vi "Test Function Generator API.vi"() -> ()   [LabVIEW 2026]
doc: "Function Generator API Tester."
uses:
  <vilib>/Utility/error.llb/DialogType.ctl
  <vilib>/Utility/error.llb/Search and Replace Pattern (string).vi
  Function Generator.lvlib
panel:
  out "Map":map{i32, dbl[]}(c390)
  in  "Stop FGEN":bool
  in  "Start":bool
  in  "amplitude":dbl=1.0 format="%0.2p"
  in  "phase":dbl format="%.2p"
  in  "frequency":dbl=10.0 format="%0.2p"
  in  "offset":dbl format="%0.2p"
  in  "Set Signal Parameters":bool
  in  "signal type":T1(ring)
  in  "Set Signal Type":bool
  out "last error":errorcluster
  in  "Show Diagram on Init":bool
  in  "Run as Singleton?":bool
  in  "Show Block Diagram":bool
  in  "Refresh Modules":bool
  out "Active Modules":string[](array[string])
  in  "Stop Module":bool
  in  "Select Module":i32(ring)=-1 caption="Select Module\nTo send Request to" items=["All"=-1]
  in  "Run New Module":bool
  in  "Hide Module Panel":bool
  in  "Show Module Panel":bool
  out "Status":string
  # "This VI tests the API for the Module."
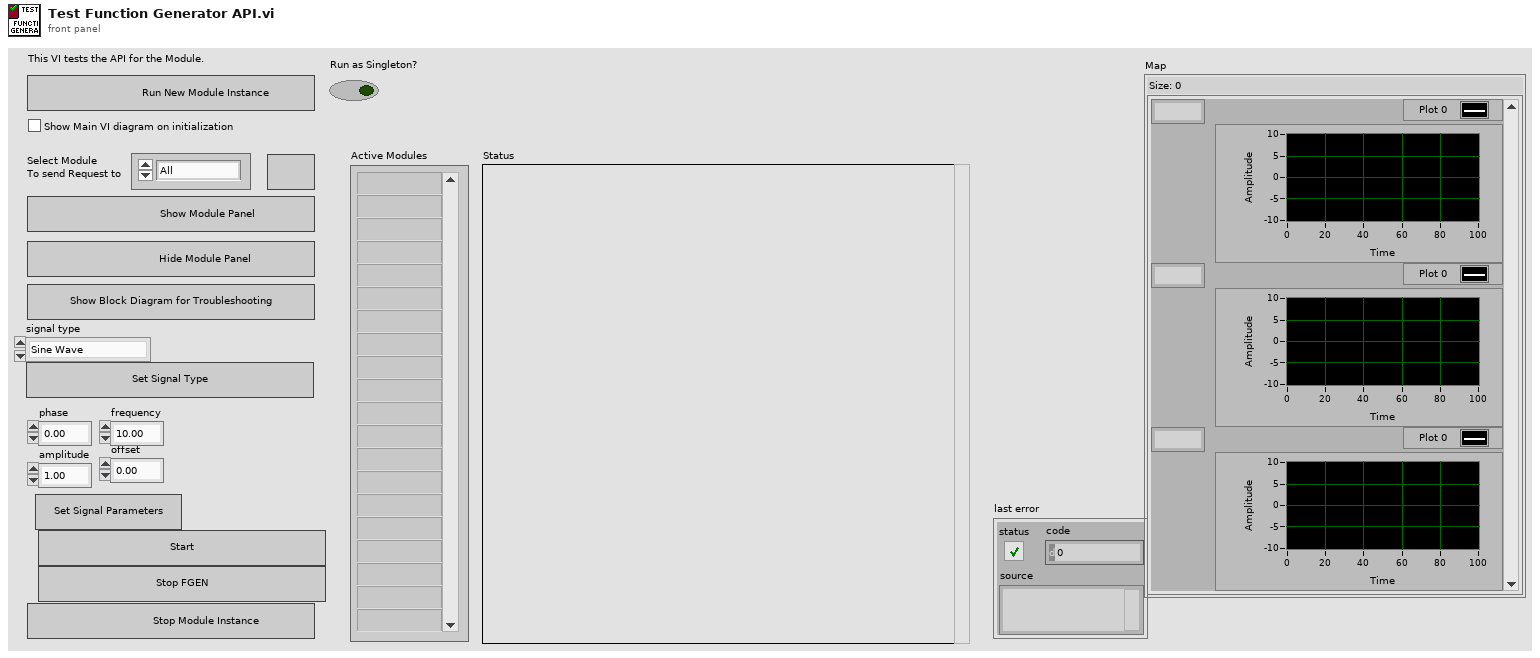
[diagram p1: front panel]
types:
  T1 = enum16{"Sine Wave", "Triangle Wave", "Square Wave", "Sawtooth Wave"}
  T2 = typedef "Function Generator.lvlib/Broadcast Events--cluster.ctl" = cluster{"Module Did Init":refnum<user-event>, "Status Updated":refnum<user-event>, "Error Reported":refnum<user-event>, "Module Did Stop":refnum<user-event>, "Update Module Execution Status":refnum<user-event>, "Waveform Updated":refnum<user-event>}
  T3 = typedef "DialogType.ctl" = u16
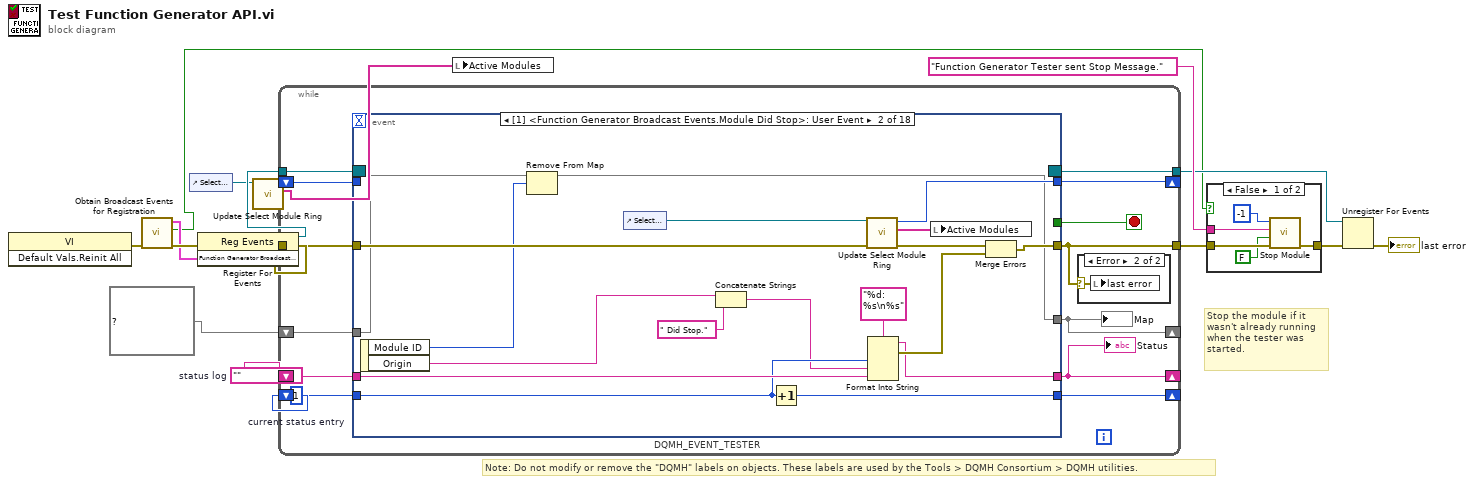
[diagram p0: block diagram]
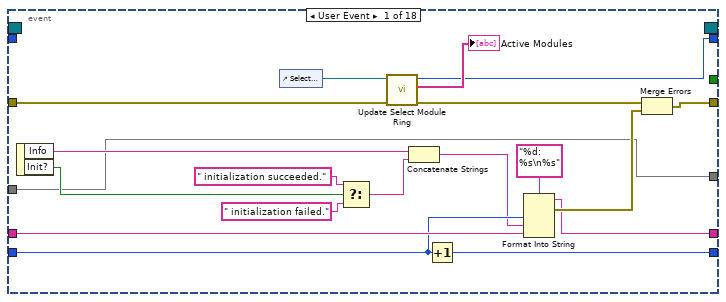
[diagram p4: hidden frame]
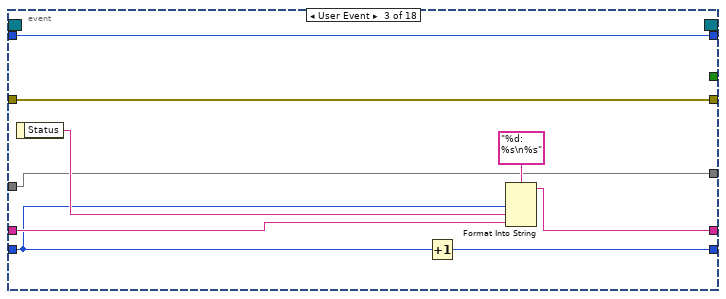
[diagram p5: hidden frame]
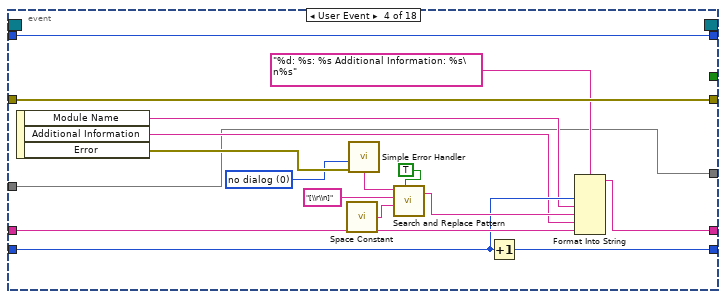
[diagram p6: hidden frame]
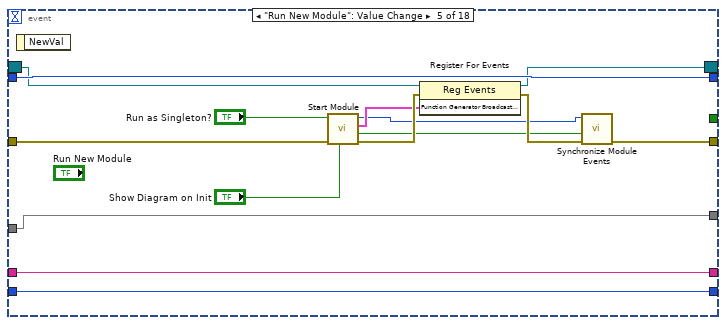
[diagram p7: hidden frame]
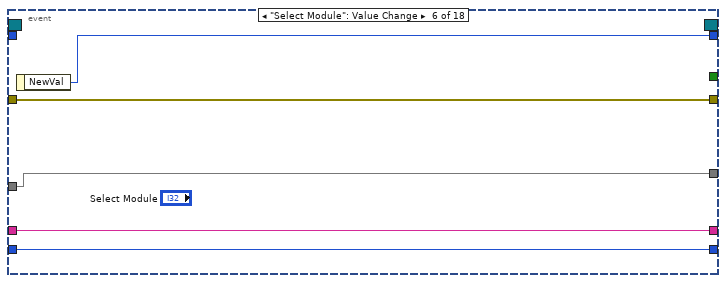
[diagram p8: hidden frame]
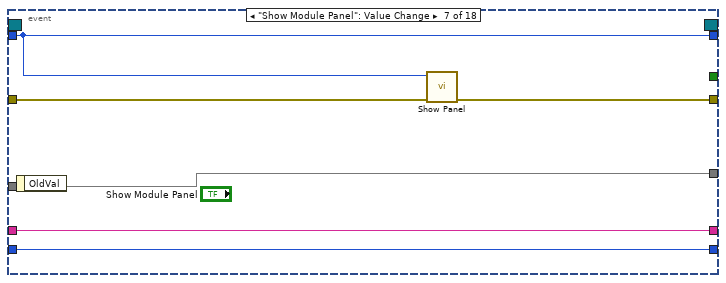
[diagram p9: hidden frame]
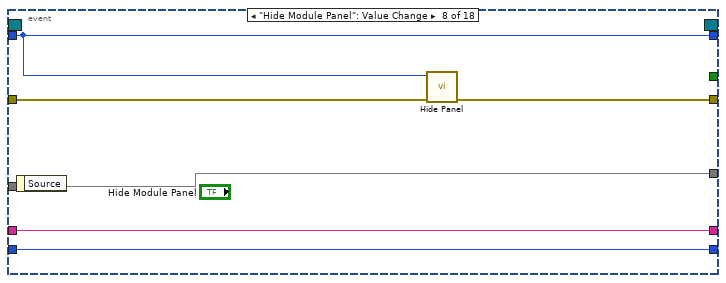
[diagram p10: hidden frame]
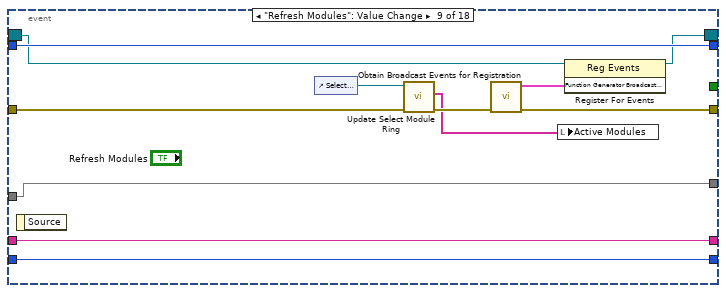
[diagram p11: hidden frame]
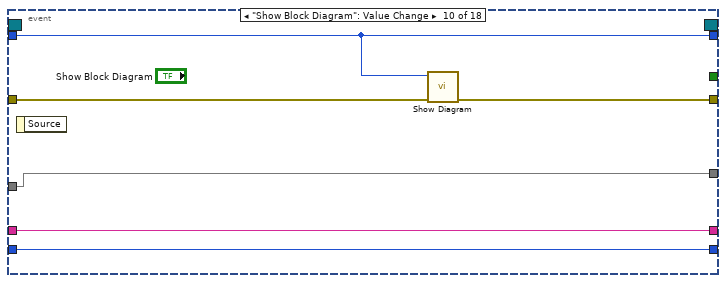
[diagram p12: hidden frame]
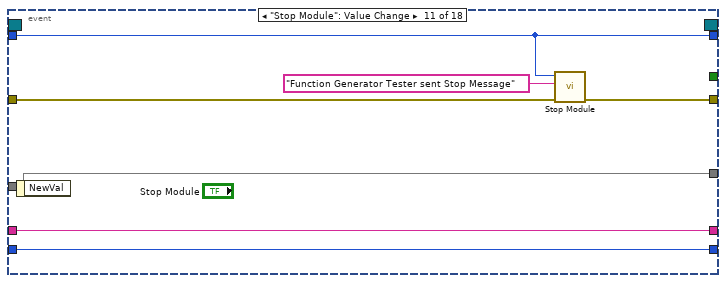
[diagram p13: hidden frame]
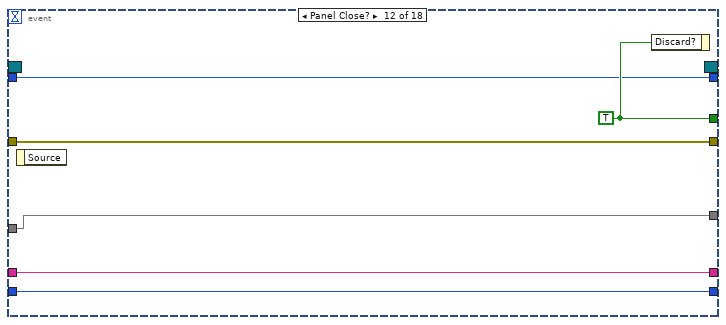
[diagram p14: hidden frame]
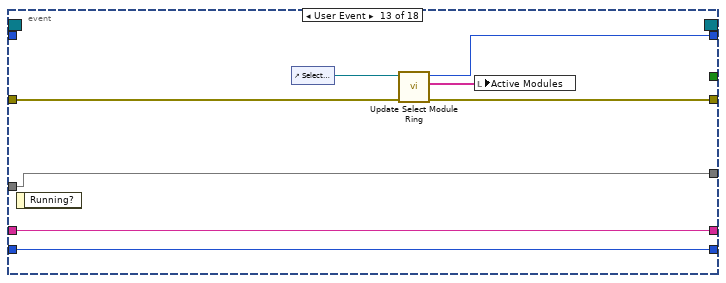
[diagram p15: hidden frame]
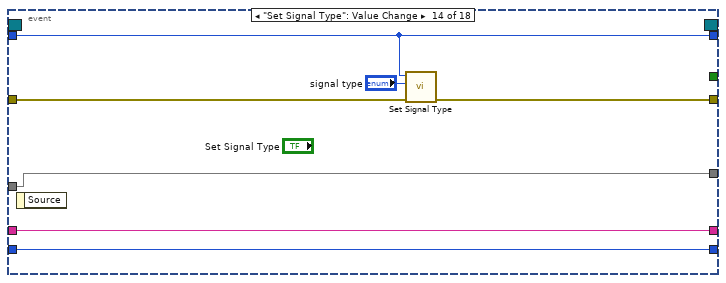
[diagram p16: hidden frame]
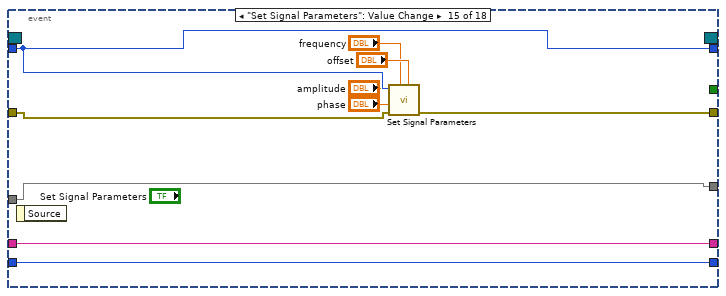
[diagram p17: hidden frame]
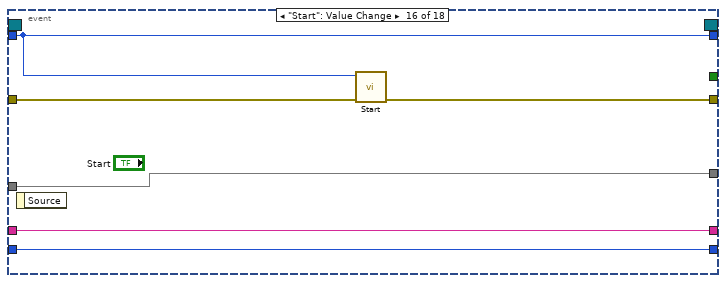
[diagram p18: hidden frame]
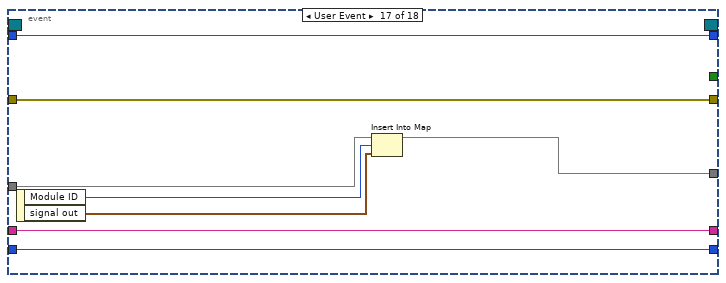
[diagram p19: hidden frame]
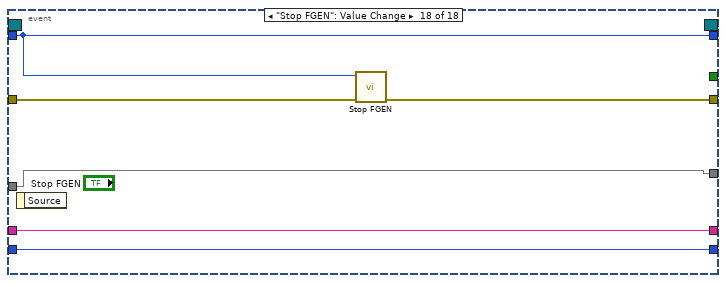
[diagram p20: hidden frame]
diagram:
  w9 = 1  # current status entry
  w10 = ""  # status log
  # "Stop the module if it wasn't already running when the tester was started."
  # "Note: Do not modify or remove the \"DQMH\" labels on objects. These labels are used by the Tools > DQMH Consortium > DQMH utilities."
  n1 = invoke on="Invoke Node" class="VI" method="Default Vals.Reinit All"() -> (error out=w15:errorcluster)  [unwired: 3 in, 2 out]
  n2 = call "Obtain Broadcast Events for Registration.vi"("error in"=w15) -> ("error out"=w14:errorcluster, "Already running?"=w5:bool, "Function Generator Broadcast Events"=w8:T2)  [unwired: 8 in]
  n3 = control-ref of="Select Module"() -> (w4:refnum<vi>)
  n4 = register-events(error in=w14, w8) -> (reference out=w11:refnum<event-registration>, error out=w16:errorcluster)  [unwired: 1 in]
  n5 = call "Update Select Module Ring.vi"("Select Module Ring Ref"=w4) -> ("Active Modules (Array)"=w2:string[], "New Module Ring Value"=w3:i32)  [unwired: 8 in, 1 out]
  n6 = while {
    tunnel: w11 -> [w28]
    tunnel: [w29] -> w13
    tunnel: w16 -> [w30]
    shift-right: [w24] -> _
    shift-left: w10 -> [w26]
    shift-right: [w25] -> _
    shift-left: w9 -> [w27]
    shift-right: [w22] -> _
    shift-left: w3 -> [w23]
    tunnel: [w21] -> w6
    shift-right: [w18] -> _
    shift-left: map{i32, dbl[]} {} ("Map") -> [w19]
    stop <- w20 stop-if-true
    n7 = event "DQMH_EVENT_TESTER" shown="[1] <Function Generator Broadcast Events.Module Did Stop>: User Event" {
      selector: w28 -> [_ _ _ _ w102 _ _ _ w131 _ _ _ _ _ _ _ _ _]
      dyn-events: [_ _ _ _ w101 _ _ _ w130 _ _ _ _ _ _ _ _ _] -> w21
      timeout: _ -> [_ _ _ _ _ _ _ _ _ _ _ _ _ _ _ _ _ _]
      tunnel: [_ _ _ _ _ _ _ _ _ _ _ w156 _ _ _ _ _ _] -> w20
      tunnel: [w47 w65 w77 w94 w106 w114 w119 w125 w136 w143 w150 w157 w164 w171 w181 w187 w196 w201] -> w29
      tunnel: w30 -> [w49 w67 w77 w94 w107 w114 w120 w126 w138 w144 w151 w157 w165 w172 w182 w188 w196 w202]
      tunnel: w27 -> [w44 w62 w70 w83 w104 w112 w117 w123 w134 w141 w148 w154 w162 w169 w179 w185 w193 w199]
      tunnel: w26 -> [w45 w63 w73 w84 w105 w113 w118 w124 w135 w142 w149 w155 w163 w170 w180 w186 w194 w200]
      tunnel: [w42 w60 w74 w82 w105 w113 w118 w124 w135 w142 w149 w155 w163 w170 w180 w186 w194 w200] -> w24
      tunnel: [w43 w61 w76 w81 w104 w112 w117 w123 w134 w141 w148 w154 w162 w169 w179 w185 w193 w199] -> w25
      tunnel: w23 -> [_ _ w71 w92 w103 _ w116 w122 w133 w140 w147 w153 _ w168 w178 w184 w195 w198]
      tunnel: [w37 w57 w71 w92 w103 w111 w116 w122 w133 w140 w147 w153 w160 w168 w178 w184 w195 w198] -> w22
      tunnel: w19 -> [w32 w53 w69 w78 w95 w110 w115 w121 w127 w139 w145 w152 w158 w166 w173 w183 w192 w197]
      tunnel: [w32 w52 w69 w78 w95 w110 w115 w121 w127 w139 w145 w152 w158 w166 w173 w183 w189 w197] -> w18
      event User Event {
        n8 = event-data() -> ("Info"=w41:string, "Init?"=w34:bool)  [unwired: 1 in]
        n9 = control-ref of="Select Module"() -> (w39:refnum<vi>)
        n10 = Select(t=" initialization succeeded.", s=w34, f=" initialization failed.") -> (s? t:f=w33:string)
        n11 = call "Update Select Module Ring.vi"("error in"=w49, "Select Module Ring Ref"=w39) -> ("error out"=w48:errorcluster, "Active Modules (Array)"=→"Active Modules":string[], "New Module Ring Value"=w37:i32)  [unwired: 7 in]
        n12 = Concatenate Strings(w41, w33) -> (w40:string)
        n13 = Increment(x=w44) -> (x+1=w43:i32)
        n14 = Format Into String(format string="%d: %s\n%s", w44, w40, w45) -> (resulting string=w42:string, error out=w50:errorcluster)  [unwired: 2 in]
        n15 = Merge Errors(w48, w50) -> (w47:errorcluster)
      }
      event User Event {
        n16 = event-data() -> ("Module ID"=w51:i32, "Origin"=w55:string)  [unwired: 1 in]
        n17 = Remove From Map(10:w51, 11:w53) -> (3:w52:map{i32, dbl[]})  [unwired: 2 out]
        n18 = control-ref of="Select Module"() -> (w59:refnum<vi>)
        n19 = Concatenate Strings(w55, " Did Stop.") -> (w54:string)
        n20 = Increment(x=w62) -> (x+1=w61:i32)
        n21 = call "Update Select Module Ring.vi"("error in"=w67, "Select Module Ring Ref"=w59) -> ("error out"=w66:errorcluster, "Active Modules (Array)"=w58:string[], "New Module Ring Value"=w57:i32)  [unwired: 7 in]
        n22 = Format Into String(format string="%d: %s\n%s", w62, w54, w63) -> (resulting string=w60:string, error out=w68:errorcluster)  [unwired: 2 in]
        n23 = local write "Active Modules"(w58) -> ()
        n24 = Merge Errors(w66, w68) -> (w65:errorcluster)
      }
      event User Event {
        n25 = event-data() -> ("Status"=w72:string)  [unwired: 1 in]
        n26 = Increment(x=w70) -> (x+1=w76:i32)
        n27 = Format Into String(format string="%d: %s\n%s", w70, w72, w73) -> (resulting string=w74:string)  [unwired: 2 in, 1 out]
      }
      event User Event {
        w85 = T3 0 items=["no dialog", "OK message", "continue or stop message", "OK message + warnings", "continue/stop + warnings"] ("type of dialog (OK msg:1)")
        n28 = event-data() -> ("Module Name"=w80:string, "Additional Information"=w79:string, "Error"=w93:errorcluster)  [unwired: 1 in]
        n29 = call <vilib>:"Space Constant.vi"() -> ("String"=w89:string)
        n30 = call <vilib>:"Simple Error Handler.vi"("type of dialog (OK msg:1)"=w85, "error in (no error)"=w93) -> ("message"=w86:string)  [unwired: 3 in, 4 out]
        n31 = call-poly <vilib>:"Search and Replace Pattern.vi"("string"=w86, "regular expression (\"\")"="[\\r\\n]" ("regular expression (\"\")"), "replace string (\"\")"=w89, "replace all? (F)"=TRUE ("replace all CR/LF with spaces")) -> ("result string"=w87:string)  [unwired: 1 in, 1 out]
        n32 = Increment(x=w83) -> (x+1=w81:i32)
        n33 = Format Into String(format string="%d: %s: %s Additional Information: %s\n%s", w83, w80, w87, w79, w84) -> (resulting string=w82:string)  [unwired: 2 in, 1 out]
      }
      event "Run New Module": Value Change {
        n34 = event-data() -> ()  [unwired: 1 in, 1 out]
        n35 = call "Start Module.vi"("Show Main VI Diagram on Init (F)"="Show Diagram on Init", "error in"=w107, "Run as Singleton? (F)"="Run as Singleton?") -> ("error out"=w108:errorcluster, "Wait for Event Sync?"=w100:bool, "Function Generator Broadcast Events"=w99:T2, "Module ID"=w96:i32)  [unwired: 4 in, 1 out]
        n36 = register-events(reference=w102, error in=w108, w99) -> (reference out=w101:refnum<event-registration>, error out=w109:errorcluster)
        n37 = call "Synchronize Module Events.vi"("error in"=w109, "Wait for Event Sync?"=w100, "Module ID in"=w96) -> ("error out"=w106:errorcluster)  [unwired: 7 in, 1 out]
      }
      event "Select Module": Value Change {
        n38 = event-data() -> ("NewVal"=w111:i32)  [unwired: 1 in]
      }
      event "Show Module Panel": Value Change {
        n39 = event-data() -> ()  [unwired: 1 in, 1 out]
        n40 = call "Show Panel.vi"("error in"=w120, "Module ID"=w116) -> ("error out"=w119:errorcluster)  [unwired: 9 in]
      }
      event "Hide Module Panel": Value Change {
        n41 = event-data() -> ()  [unwired: 1 in, 1 out]
        n42 = call "Hide Panel.vi"("error in"=w126, "Module ID"=w122) -> ("error out"=w125:errorcluster)  [unwired: 9 in]
      }
      event "Refresh Modules": Value Change {
        n43 = event-data() -> ()  [unwired: 1 in, 1 out]
        n44 = control-ref of="Select Module"() -> (w132:refnum<vi>)
        n45 = call "Update Select Module Ring.vi"("error in"=w138, "Select Module Ring Ref"=w132) -> ("error out"=w137:errorcluster, "Active Modules (Array)"=w128:string[])  [unwired: 7 in, 1 out]
        n46 = call "Obtain Broadcast Events for Registration.vi"("error in"=w137) -> ("error out"=w136:errorcluster, "Function Generator Broadcast Events"=w129:T2)  [unwired: 8 in, 1 out]
        n47 = local write "Active Modules"(w128) -> ()
        n48 = register-events(reference=w131, w129) -> (reference out=w130:refnum<event-registration>)  [unwired: 1 in, 1 out]
      }
      event "Show Block Diagram": Value Change {
        n49 = event-data() -> ()  [unwired: 1 in, 1 out]
        n50 = call "Show Diagram.vi"("error in"=w144, "Module ID"=w140) -> ("error out"=w143:errorcluster)  [unwired: 9 in]
      }
      event "Stop Module": Value Change {
        n51 = event-data() -> ()  [unwired: 1 in, 1 out]
        n52 = call "Stop Module.vi"("error in"=w151, "Origin"="Function Generator Tester sent Stop Message", "Module ID"=w147) -> ("error out"=w150:errorcluster)  [unwired: 8 in]
      }
      event Panel Close? {
        w156 = TRUE ("Discard?")
        n53 = event-data() -> ()  [unwired: 1 in, 1 out]
        n54 = event-data ("Event Filter Node")("Discard?"=w156) -> ()  [unwired: 1 in, 1 out]
      }
      event User Event {
        n55 = event-data() -> ()  [unwired: 1 in, 1 out]
        n56 = control-ref of="Select Module"() -> (w161:refnum<vi>)
        n57 = call "Update Select Module Ring.vi"("error in"=w165, "Select Module Ring Ref"=w161) -> ("error out"=w164:errorcluster, "Active Modules (Array)"=w159:string[], "New Module Ring Value"=w160:i32)  [unwired: 7 in]
        n58 = local write "Active Modules"(w159) -> ()
      }
      event "Set Signal Type": Value Change {
        n59 = event-data() -> ()  [unwired: 1 in, 1 out]
        n60 = call "Set Signal Type.vi"("error in"=w172, "signal type"="signal type", "Module ID"=w168) -> ("error out"=w171:errorcluster)  [unwired: 8 in]
      }
      event "Set Signal Parameters": Value Change {
        n61 = event-data() -> ()  [unwired: 1 in, 1 out]
        n62 = call "Set Signal Parameters.vi"("offset"="offset", "frequency"="frequency", "error in"=w182, "phase"="phase", "amplitude"="amplitude", "Module ID"=w178) -> ("error out"=w181:errorcluster)  [unwired: 5 in]
      }
      event "Start": Value Change {
        n63 = event-data() -> ()  [unwired: 1 in, 1 out]
        n64 = call "Start.vi"("error in"=w188, "Module ID"=w184) -> ("error out"=w187:errorcluster)  [unwired: 9 in]
      }
      event User Event {
        n65 = event-data() -> ("Module ID"=w191:i32, "signal out"=w190:waveform(dbl))  [unwired: 1 in]
        n66 = Insert Into Map(map in=w192, key=w191, value=w190) -> (map out=w189:map{i32, dbl[]})  [unwired: 2 out]
      }
      event "Stop FGEN": Value Change {
        n67 = event-data() -> ()  [unwired: 1 in, 1 out]
        n68 = call "Stop FGEN.vi"("error in"=w202, "Module ID"=w198) -> ("error out"=w201:errorcluster)  [unwired: 9 in]
      }
    }
    "Status" <- w24
    "Map" <- w18
    n69 = case shown="Error" w29 {
      selector: w29 -> [_ w31]
      frame No Error {
      }
      frame Error {
        n70 = local write "last error"(w31) -> ()
      }
    }
  }
  n71 = local write "Active Modules"(w2) -> ()
  n72 = case shown="False" w5 {
    tunnel: [w207 w208] -> w17
    tunnel: "Function Generator Tester sent Stop Message." ("Origin") -> [w205 _]
    tunnel: w13 -> [w206 w208]
    frame False {
      n73 = call "Stop Module.vi"("error in"=w206, "Wait for Module to stop? (F)"=FALSE ("Wait for Module to stop?"), "Origin"=w205, "Module ID"=-1 ("Stop all")) -> ("error out"=w207:errorcluster)  [unwired: 7 in]
    }
    frame True {
    }
  }
  n74 = Unregister For Events(event registration refnum=w6, error in=w17) -> (error out=→"last error":errorcluster)
